vi "Start Reader.vi"(8 "error in (no error)":errorcluster, 11 "XNET_CAN_RW in":refnum<class "XNET CAN RW.lvclass">) -> (0 "error out":errorcluster, 3 "XNET_CAN_RW out":refnum<class "XNET CAN RW.lvclass">)   [LabVIEW 2021, in "XNET CAN RW.lvclass"]
uses:
  XNET CAN RW.lvclass
  C:/Program Files/National Instruments/LabVIEW 2021/vi.lib/CIF Foundation/CIF CAN RW Core/CAN_RW_CORE.lvclass
  <vilib>/CIF Foundation/CIF CAN RW Core/CAN_RW_CORE.lvclass/CAN_RW_CORE.ctl
  <vilib>/CIF Foundation/CIF CAN RW Core/typedef/CAN Interface Mode.ctl
  XNET CAN RW.lvclass/XNET CAN RW.ctl
  <vilib>/CIF Foundation/CIF CAN RW Core/Accessors/Read Interface.vi
  <vilib>/CIF Foundation/CIF CAN RW Core/Accessors/Read Port Configuration.vi
  <vilib>/CIF Foundation/CIF CAN RW Core/Accessors/Write CAN Interface Mode.vi
  <vilib>/xnet/xnet.llb/XNET Create Session (Frame Input Stream).vi
  <resource>/objmgr/xnet.rc
  <vilib>/CIF Foundation/CIF CAN RW Core/CAN_RW_CORE.lvclass
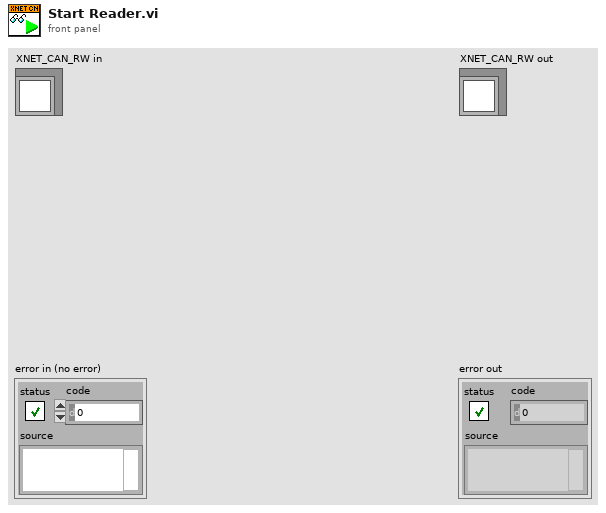
[diagram p1: front panel]
types:
  T1 = typedef "CAN_RW_CORE.lvclass/CAN Port Configuration.ctl" = cluster{"Mode":T2, "Baud Rate":u64, "Temination On":bool, "Subordinate":bool, "Echo TX":bool, "FD Config":T3}
  T2 = typedef "CAN_RW_CORE.lvclass/CAN Mode.ctl" = enum16{"CAN 2.0", "CAN FD"}
  T3 = typedef "CAN_RW_CORE.lvclass/FD Config.ctl" = cluster{"FD Baud Rate":u64, "ISO Mode":bool, "BRS Enabled":bool}
  T4 = typedef "CAN_RW_CORE.lvclass/CAN Interface Mode.ctl" = enum16{"Unknown", "CAN 2.0", "CAN FD", "CAN FD BRS"}
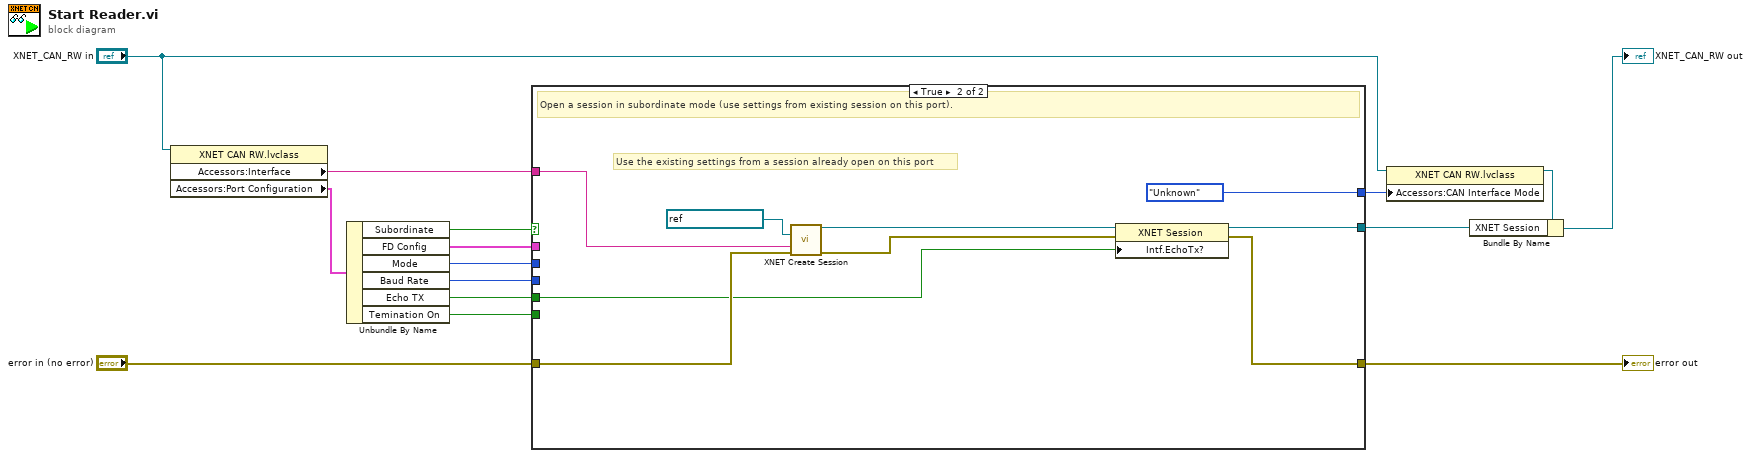
[diagram p0: block diagram]
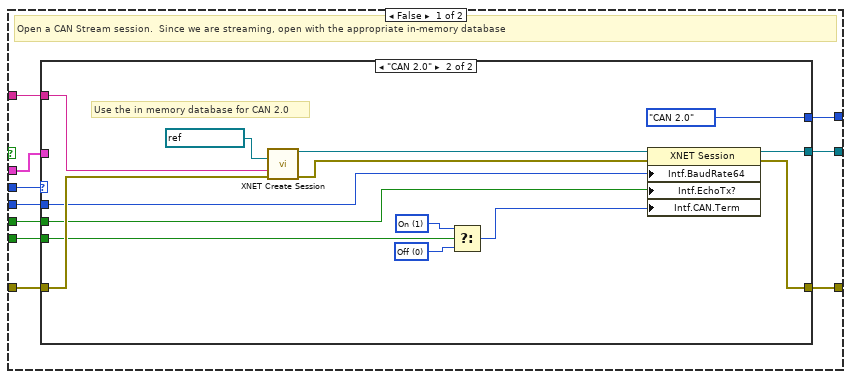
[diagram p2: hidden frame]
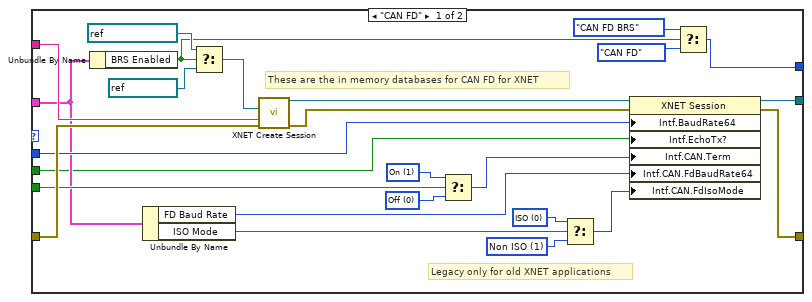
[diagram p3: hidden frame]
diagram:
  n1 = property class="XNET CAN RW.lvclass"(reference="XNET_CAN_RW in") -> ("Accessors:Interface"=w4:string, "Accessors:Port Configuration"=w5:T1)  [unwired: 1 in, 2 out]
  n2 = Unbundle By Name(w5) -> ("Subordinate"=w10:bool, "FD Config"=w13:T3, "Mode"=w12:T2, "Baud Rate"=w14:u64, "Echo TX"=w6:bool, "Temination On"=w7:bool)
  n3 = case shown="True" w10 {
    tunnel: w4 -> [w25 w73]
    tunnel: "error in (no error)" -> [w24 w72]
    tunnel: w14 -> [w23 _]
    tunnel: w7 -> [w22 _]
    tunnel: w13 -> [w21 _]
    tunnel: w12 -> [w20 _]
    tunnel: [w19 w69] -> w9
    tunnel: [w18 w67] -> w8
    tunnel: w6 -> [w17 w66]
    tunnel: [w16 CAN_Interface_Mode."Unknown" ("CAN Interface Mode")] -> w2
    frame False {
      # "Open a CAN Stream session.  Since we are streaming, open with the appropriate in-memory database"
      n4 = case shown="\"CAN 2.0\"" w20 {
        tunnel: w25 -> [w50 w64]
        tunnel: w24 -> [w49 w63]
        tunnel: w23 -> [w41 w58]
        tunnel: w22 -> [w42 w59]
        tunnel: w21 -> [w39 _]
        tunnel: [w34 w56] -> w18
        tunnel: [w33 w55] -> w19
        tunnel: w17 -> [w30 w53]
        tunnel: [w28 CAN_Interface_Mode."CAN 2.0" ("CAN Interface Mode")] -> w16
        frame "CAN FD" {
          w36 = u32 1 items=["ISO", "Non ISO", "ISO Legacy"] ("Interface:CAN:FD ISO Mode")
          w37 = u32 0 items=["ISO", "Non ISO", "ISO Legacy"] ("Interface:CAN:FD ISO Mode")
          w40 = u32 0 items=["Off", "On"] ("Interface:CAN:Termination")
          w44 = u32 1 items=["Off", "On"] ("Interface:CAN:Termination")
          # "These are the in memory databases for CAN FD for XNET"
          # "Legacy only for old XNET applications"
          n5 = Unbundle By Name(w39) -> ("BRS Enabled"=w26:bool)
          n6 = Unbundle By Name(w39) -> ("FD Baud Rate"=w32:u64, "ISO Mode"=w38:bool)
          n7 = Select(t=refnum<k21> ":can_fd_brs:" ("cluster (:memory:)"), s=w26, f=refnum<k21> ":can_fd:" ("cluster (:memory:)")) -> (s? t:f=w46:refnum<k21>)
          n8 = call-poly <vilib>:"XNET Create Session.vi"("cluster (:memory:)"=w46, "interface"=w50, "error in (no error)"=w49) -> ("session out"=w45:refnum<k21>, "error out"=w43:errorcluster)  [unwired: 11 in]
          n9 = Select(t=w44, s=w42, f=w40) -> (s? t:f=w31:u32)
          n10 = Select(t=w37, s=w38, f=w36) -> (s? t:f=w35:u32)
          n11 = property class="XNET Session"(reference=w45, error in=w43, "Intf.BaudRate64"=w41, "Intf.EchoTx?"=w30, "Intf.CAN.Term"=w31, "Intf.CAN.FdBaudRate64"=w32, "Intf.CAN.FdIsoMode"=w35) -> (reference out=w33:refnum<k21>, error out=w34:errorcluster)
          n12 = Select(t=CAN_Interface_Mode."CAN FD BRS" ("CAN Interface Mode"), s=w26, f=CAN_Interface_Mode."CAN FD" ("CAN Interface Mode")) -> (s? t:f=w28:T4)
        }
        frame "CAN 2.0" {
          w57 = u32 0 items=["Off", "On"] ("Interface:CAN:Termination")
          w61 = u32 1 items=["Off", "On"] ("Interface:CAN:Termination")
          # "Use the in memory database for CAN 2.0"
          n13 = call-poly <vilib>:"XNET Create Session.vi"("cluster (:memory:)"=refnum<k21> ":memory:", "interface"=w64, "error in (no error)"=w63) -> ("session out"=w62:refnum<k21>, "error out"=w60:errorcluster)  [unwired: 11 in]
          n14 = Select(t=w61, s=w59, f=w57) -> (s? t:f=w54:u32)
          n15 = property class="XNET Session"(reference=w62, error in=w60, "Intf.BaudRate64"=w58, "Intf.EchoTx?"=w53, "Intf.CAN.Term"=w54) -> (reference out=w55:refnum<k21>, error out=w56:errorcluster)
        }
      }
    }
    frame True {
      # "Use the existing settings from a session already open on this port"
      # "Open a session in subordinate mode (use settings from existing session on this port)."
      n16 = call-poly <vilib>:"XNET Create Session.vi"("cluster (:memory:)"=refnum<k21> ":subordinate:", "interface"=w73, "error in (no error)"=w72) -> ("session out"=w70:refnum<k21>, "error out"=w68:errorcluster)  [unwired: 11 in]
      n17 = property class="XNET Session"(reference=w70, error in=w68, "Intf.EchoTx?"=w66) -> (reference out=w69:refnum<k21>, error out=w67:errorcluster)
    }
  }
  "error out" <- w8
  n18 = property class="XNET CAN RW.lvclass"(reference="XNET_CAN_RW in", "Accessors:CAN Interface Mode"=w2) -> (reference out=w1:refnum<class "XNET CAN RW.lvclass">)  [unwired: 1 in, 1 out]
  n19 = Bundle By Name(cluster=w1, "XNET Session"=w9) -> (→"XNET_CAN_RW out":refnum<class "XNET CAN RW.lvclass">)
